vi "Stimulus.GetStatusInfo.vi"(8 "error in (no error)":errorcluster, 10 "Cluster":T1={"NIVS.BaseLogPath"=path "", "NIVS.SystemDefinitionFile"=path "", "NIVS.Events"={"SequenceEvent"=refnum, "SystemChangeEvent"=refnum, "WorkspaceEvent"=refnum}, "NIVS.SequenceState"=enum."Idle", "NIVS.GatewayIPAddress"="", "NIVS.DataLogSpecRef"=refnum, "NIVS.DataLogManagerRef"=refnum, "NIVS.LogSessionGUID"="", "NIVS.WorkspaceManager"=refnum, "NIVS.Deployed"=FALSE, "NIVS.ProfileRef"=refnum, "NIVS.ProfileCallback"=refnum, "NIVS.SystemStateRefs"={"CustDatRef"=refnum, "EvtRef"=refnum, "Target State User Event"=refnum}, "UI.Abort"=refnum, "UI.Pause"=refnum, "UI.EnableLogging"=refnum, "UI.Start"=refnum, "UI.LogChannels"=refnum, "UI.StartIteration"=refnum, "UI.StartStep"=refnum, "UI.Sequence"=refnum, "UI.PreviewMode"=refnum, "UI.Graph"=refnum, "UI.BaseFileName"=refnum, "UI.Profiles"=refnum, "UI.CurrentStep"=refnum, "UI.CurrentIteration"=refnum, "UI.TotalIterations"=refnum, "Sequence.AbortChannel"="", "Sequence.StepInfoChannel"="", "Sequence.Iterations"=0, "Sequence.IterationInfoChannel"="", "Sequence.#ofColumns"=0, "Events.State"=refnum, "Events.Test Result"=refnum, "Events.Progress"=refnum, "INI.Settings"={"Build Location"=path "C:/Simple Sequence Editor/SequenceRepo", "LoggingLocation"=path ""}, "UI.Skip"=refnum, "Sequence.SkipChannel"="", "Restart.Path"=path "", "UI.Duration"=refnum, "Sequence.DurationChannel"=""}, 11 "Commands":string[](array[string])) -> (0 "error out":errorcluster, 3 "Commands out":string[](array[string]))   [LabVIEW 2015, in "Simple Sequence Tools - Execution.lvlib"]
uses:
  Simple Sequence Tools - Execution.lvlib
  Types/Main.StateVariables.ctl
  Types/Execute.UserEventRefs.ctl
  <vilib>/NI Veristand/Execution/Workspace/SystemStateRegEventRef.ctl
  <vilib>/NI Veristand/Execution/Workspace/Target State Info.ctl
  <vilib>/NI Veristand/Execution/Workspace/Target State.ctl
  Types/Execution.SequenceState.ctl
  <vilib>/NI Veristand/Execution/DataLogging/DataLoggingSpecification Ref.ctl
  NationalInstruments.VeriStand.ClientAPI
  <vilib>/NI Veristand/Execution/DataLogging/IDataLogging Ref.ctl
  <vilib>/NI Veristand/Execution/Workspace/WorkspaceAPI.ctl
  NationalInstruments.VeriStand.RealTimeSequenceDefinitionApi
  <vilib>/NI Veristand/Execution/Workspace/SystemStateEventRef.ctl
  Shared/Types/INI.Settings.ctl
  <vilib>/NI Veristand/Execution/Workspace/NI VeriStand - Get Single Channel Value.vi
  <vilib>/NI Veristand/Execution/Workspace/NI_VS Workspace ExecutionAPI.lvlib
  <vilib>/NI Veristand/Execution/DataLogging/NI_VS Data Logging API.lvlib
  Shared/Simple Sequence Tools - Shared.lvlib
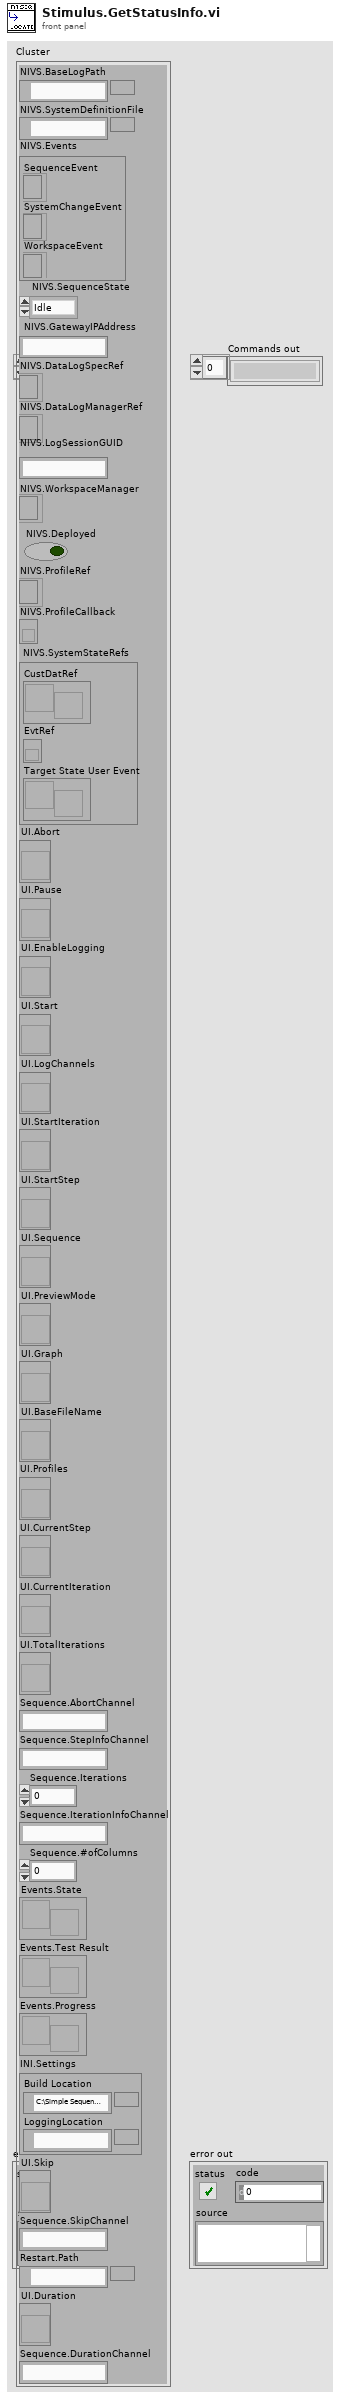
[diagram p1: front panel]
types:
  T1 = typedef "Simple Sequence Tools - Execution.lvlib/Main.StateVariables.ctl" = cluster{"NIVS.BaseLogPath":path, "NIVS.SystemDefinitionFile":path, "NIVS.Events":T2, "NIVS.SequenceState":T4, "NIVS.GatewayIPAddress":string, "NIVS.DataLogSpecRef":T5, "NIVS.DataLogManagerRef":T6, "NIVS.LogSessionGUID":string, "NIVS.WorkspaceManager":T7, "NIVS.Deployed":bool, "NIVS.ProfileRef":refnum<k24>, "NIVS.ProfileCallback":refnum<k27>, "NIVS.SystemStateRefs":T8, "UI.Abort":refnum<vi>, "UI.Pause":refnum<vi>, "UI.EnableLogging":refnum<vi>, "UI.Start":refnum<vi>, "UI.LogChannels":refnum<vi>, "UI.StartIteration":refnum<vi>, "UI.StartStep":refnum<vi>, "UI.Sequence":refnum<vi>, "UI.PreviewMode":refnum<vi>, "UI.Graph":refnum<vi>, "UI.BaseFileName":refnum<vi>, "UI.Profiles":refnum<vi>, "UI.CurrentStep":refnum<vi>, "UI.CurrentIteration":refnum<vi>, "UI.TotalIterations":refnum<vi>, "Sequence.AbortChannel":string, "Sequence.StepInfoChannel":string, "Sequence.Iterations":u32, "Sequence.IterationInfoChannel":string, "Sequence.#ofColumns":i32, "Events.State":refnum<user-event>, "Events.Test Result":refnum<user-event>, "Events.Progress":refnum<user-event>, "INI.Settings":T9, "UI.Skip":refnum<vi>, "Sequence.SkipChannel":string, "Restart.Path":path, "UI.Duration":refnum<vi>, "Sequence.DurationChannel":string}
  T2 = typedef "Simple Sequence Tools - Execution.lvlib/Execute.UserEventRefs.ctl" = cluster{"SequenceEvent":refnum<event-registration>, "SystemChangeEvent":T3, "WorkspaceEvent":refnum<event-registration>}
  T3 = typedef "NI_VS Workspace ExecutionAPI.lvlib/SystemStateRegEventRef.ctl" = refnum<event-registration>
  T4 = typedef "Simple Sequence Tools - Execution.lvlib/Execution.SequenceState.ctl" = enum16{"Idle", "Initializing", "Running", "Paused", "Finalizing", "Complete"}
  T5 = typedef "NI_VS Data Logging API.lvlib/DataLoggingSpecification Ref.ctl" = refnum<k24>
  T6 = typedef "NI_VS Data Logging API.lvlib/IDataLogging Ref.ctl" = refnum<k24>
  T7 = typedef "NI_VS Workspace ExecutionAPI.lvlib/WorkspaceAPI.ctl" = refnum<k24>
  T8 = typedef "NI_VS Workspace ExecutionAPI.lvlib/SystemStateEventRef.ctl" = cluster{"CustDatRef":refnum<user-event>, "EvtRef":refnum<k27>, "Target State User Event":refnum<user-event>}
  T9 = typedef "Simple Sequence Tools - Shared.lvlib/INI.Settings.ctl" = cluster{"Build Location":path, "LoggingLocation":path}
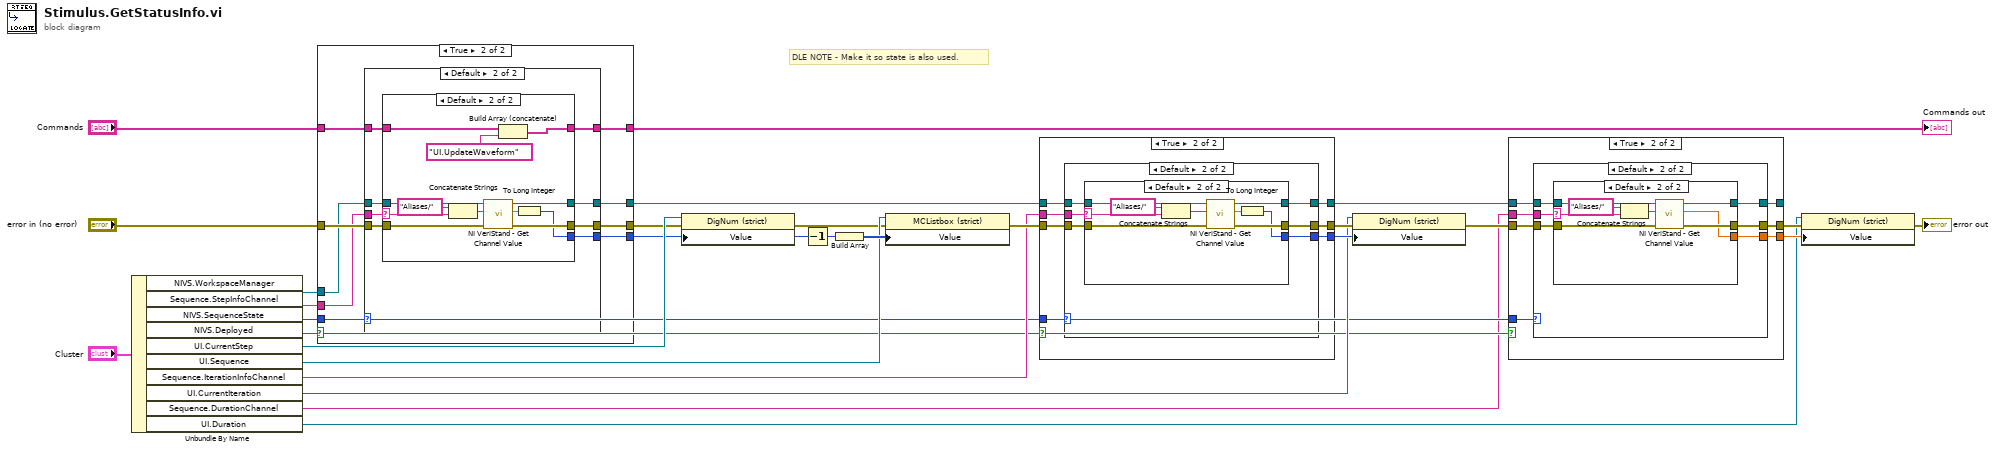
[diagram p0: block diagram]
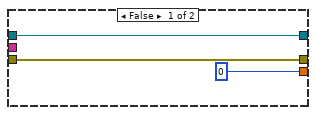
[diagram p2: hidden frame]
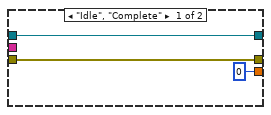
[diagram p3: hidden frame]
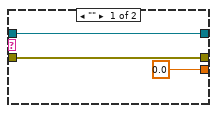
[diagram p4: hidden frame]
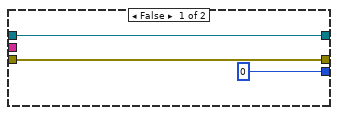
[diagram p5: hidden frame]
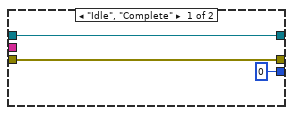
[diagram p6: hidden frame]
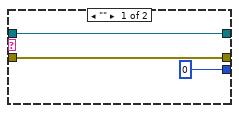
[diagram p7: hidden frame]
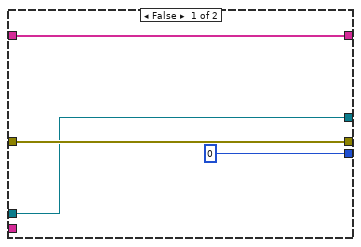
[diagram p8: hidden frame]
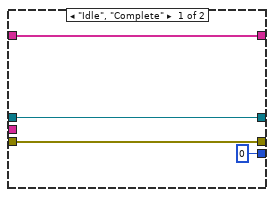
[diagram p9: hidden frame]
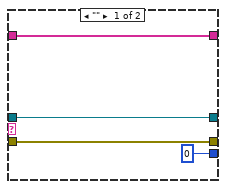
[diagram p10: hidden frame]
diagram:
  # "DLE NOTE - Make it so state is also used."
  n1 = Unbundle By Name("Cluster") -> ("NIVS.WorkspaceManager"=w20:T7, "Sequence.StepInfoChannel"=w22:string, "NIVS.SequenceState"=w5:T4, "NIVS.Deployed"=w4:bool, "UI.CurrentStep"=w17:refnum<vi>, "UI.Sequence"=w18:refnum<vi>, "Sequence.IterationInfoChannel"=w27:string, "UI.CurrentIteration"=w11:refnum<vi>, "Sequence.DurationChannel"=w3:string, "UI.Duration"=w1:refnum<vi>)
  n2 = case shown="True" w4 {
    tunnel: w20 -> [w29 w39]
    tunnel: "error in (no error)" -> [w32 w41]
    tunnel: [w32 w40] -> w15
    tunnel: w22 -> [_ w37]
    tunnel: [0 w38] -> w14
    tunnel: "Commands" -> [w30 w36]
    tunnel: [w30 w35] -> w25
    tunnel: [w29 w34] -> w26
    tunnel: w5 -> [_ w33]
    frame False {
    }
    frame True {
      n3 = case shown="Default" w33 {
        tunnel: w41 -> [w43 w53]
        tunnel: [w43 w52] -> w40
        tunnel: w39 -> [w44 w51]
        tunnel: [0 w50] -> w38
        tunnel: w37 -> [_ w49]
        tunnel: w36 -> [w45 w48]
        tunnel: [w45 w47] -> w35
        tunnel: [w44 w46] -> w34
        frame "Idle", "Complete" {
        }
        frame Default {
          n4 = case shown="Default" w49 {
            selector: w49 -> [_ w59]
            tunnel: w53 -> [w57 w69]
            tunnel: [w57 w68] -> w52
            tunnel: w51 -> [w54 w67]
            tunnel: [0 w65] -> w50
            tunnel: w48 -> [w55 w63]
            tunnel: [w55 w62] -> w47
            tunnel: [w54 w61] -> w46
            frame "" {
            }
            frame Default {
              n5 = Concatenate Strings("Aliases/" ("string"), w59) -> (w58:string)
              n6 = call-poly <vilib>:"NI VeriStand - Get Channel Value.vi"("error in (no error)"=w69, "Channel"=w58, "WorkspaceManager in"=w67) -> ("error out"=w68:errorcluster, "Value"=w66:dbl, "WorkspaceManager out"=w61:T7)  [unwired: 6 in]
              n7 = Build Array (concatenate)(w63, "UI.UpdateWaveform") -> (w62:string[])
              n8 = To Long Integer(number=w66) -> (32bit integer=w65:i32)
            }
          }
        }
      }
    }
  }
  "Commands out" <- w25
  n9 = property class="DigNum (strict)"(reference=w17, error in=w15, "Value"=w14) -> (error out=w16:errorcluster)  [unwired: 1 out]
  n10 = Decrement(x=w14) -> (x-1=w10:i32)
  n11 = Build Array(w10) -> (w23:i32[])
  n12 = property class="MCListbox (strict)"(reference=w18, error in=w16, "Value"=w23) -> (error out=w28:errorcluster)  [unwired: 1 out]
  n13 = case shown="True" w4 {
    tunnel: w26 -> [w70 w77]
    tunnel: w28 -> [w72 w79]
    tunnel: [w72 w78] -> w13
    tunnel: w27 -> [_ w75]
    tunnel: [0 w76] -> w12
    tunnel: w5 -> [_ w74]
    tunnel: [w70 w73] -> w2
    frame False {
    }
    frame True {
      n14 = case shown="Default" w74 {
        tunnel: w79 -> [w82 w88]
        tunnel: [w82 w87] -> w78
        tunnel: w77 -> [w80 w86]
        tunnel: [0 w85] -> w76
        tunnel: w75 -> [_ w84]
        tunnel: [w80 w83] -> w73
        frame "Idle", "Complete" {
        }
        frame Default {
          n15 = case shown="Default" w84 {
            selector: w84 -> [_ w93]
            tunnel: w88 -> [w91 w100]
            tunnel: [w91 w99] -> w87
            tunnel: w86 -> [w89 w98]
            tunnel: [0 w96] -> w85
            tunnel: [w89 w95] -> w83
            frame "" {
            }
            frame Default {
              n16 = Concatenate Strings("Aliases/" ("string"), w93) -> (w92:string)
              n17 = call-poly <vilib>:"NI VeriStand - Get Channel Value.vi"("error in (no error)"=w100, "Channel"=w92, "WorkspaceManager in"=w98) -> ("error out"=w99:errorcluster, "Value"=w97:dbl, "WorkspaceManager out"=w95:T7)  [unwired: 6 in]
              n18 = To Long Integer(number=w97) -> (32bit integer=w96:i32)
            }
          }
        }
      }
    }
  }
  n19 = property class="DigNum (strict)"(reference=w11, error in=w13, "Value"=w12) -> (error out=w9:errorcluster)  [unwired: 1 out]
  n20 = case shown="True" w4 {
    tunnel: w2 -> [w101 w108]
    tunnel: w9 -> [w103 w110]
    tunnel: [w103 w109] -> w8
    tunnel: w3 -> [_ w106]
    tunnel: [0 w107] -> w6
    tunnel: w5 -> [_ w105]
    tunnel: [w101 w104] -> _
    frame False {
    }
    frame True {
      n21 = case shown="Default" w105 {
        tunnel: w110 -> [w113 w119]
        tunnel: [w113 w118] -> w109
        tunnel: w108 -> [w111 w117]
        tunnel: [0 w116] -> w107
        tunnel: w106 -> [_ w115]
        tunnel: [w111 w114] -> w104
        frame "Idle", "Complete" {
        }
        frame Default {
          n22 = case shown="Default" w115 {
            selector: w115 -> [_ w124]
            tunnel: w119 -> [w122 w130]
            tunnel: [w122 w129] -> w118
            tunnel: w117 -> [w120 w128]
            tunnel: [0.0 w126] -> w116
            tunnel: [w120 w127] -> w114
            frame "" {
            }
            frame Default {
              n23 = Concatenate Strings("Aliases/" ("string"), w124) -> (w123:string)
              n24 = call-poly <vilib>:"NI VeriStand - Get Channel Value.vi"("error in (no error)"=w130, "Channel"=w123, "WorkspaceManager in"=w128) -> ("error out"=w129:errorcluster, "Value"=w126:dbl, "WorkspaceManager out"=w127:T7)  [unwired: 6 in]
            }
          }
        }
      }
    }
  }
  n25 = property class="DigNum (strict)"(reference=w1, error in=w8, "Value"=w6) -> (error out=→"error out":errorcluster)  [unwired: 1 out]
